vi "add channel to configuration.vi"(8 "error in":errorcluster, 10 "Modbus Module Channel.lvclass":refnum<class "Modbus Module Channel.lvclass">, 11 "Modbus Slave configuration in":refnum<class "Modbus Module configuration.lvclass">) -> (0 "error out":errorcluster, 3 "Modbus Slave configuration out":refnum<class "Modbus Module configuration.lvclass">)   [LabVIEW 2015, in "Modbus Module configuration.lvclass"]
doc: "Attempt to add Channel Input to Configuration's channel list.Channel will not be added if one with the same name already exists.\n\nPlatypus Framework 1.0.1.65\nNI Systems Engineering - National Instruments"
uses:
  Modbus Module configuration.lvclass
  module channel/Modbus Module Channel.lvclass
  <vilib>/NI/Tag Bus/tag/tag descriptor.lvclass/tag descriptor.ctl
  Modbus Module configuration.lvclass/Modbus Module configuration.ctl
  <vilib>/NI/Tag Bus/tag/tag descriptor.lvclass
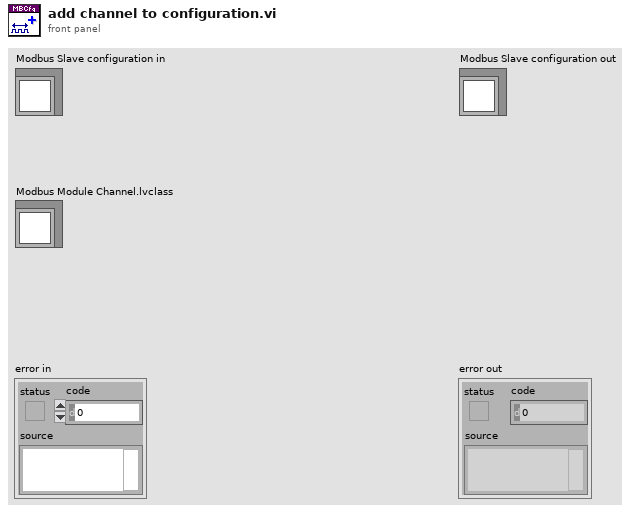
[diagram p1: front panel]
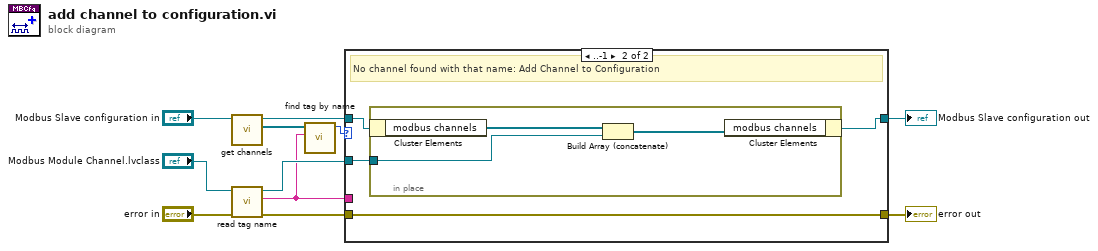
[diagram p0: block diagram]
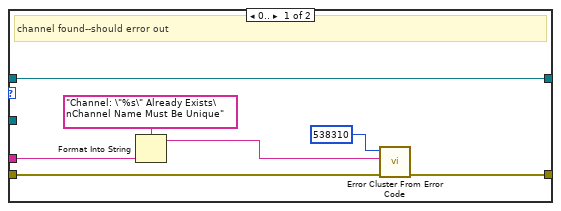
[diagram p2: hidden frame]
diagram:
  n1 = call-dynamic "get channels.vi"("Modbus Slave configuration in"="Modbus Slave configuration in") -> ("channels"=w5:refnum<class "TBM channel.lvclass">[], "Modbus Slave configuration out"=w11:refnum<class "Modbus Module configuration.lvclass">)  [unwired: 9 in]
  n2 = call <vilib>:"read tag name.vi"("error in"="error in", "system tag in"="Modbus Module Channel.lvclass") -> ("error out"=w2:errorcluster, "name"=w3:string, "system tag out"=w10:refnum<class "Modbus Module Channel.lvclass">)  [unwired: 7 in]
  n3 = call <vilib>:"find tag by name.vi"("name"=w3, "tags in"=w5) -> ("index"=w4:i32)  [unwired: 9 in]
  n4 = case shown="..-1" w4 {
    tunnel: [w18 w21] -> w8
    tunnel: w3 -> [w13 _]
    tunnel: w2 -> [w16 w21]
    tunnel: w11 -> [w15 w20]
    tunnel: w10 -> [_ w22]
    tunnel: [w15 w19] -> w7
    frame 0.. {
      # "channel found--should error out"
      n5 = Format Into String(format string="Channel: \"%s\" Already Exists\nChannel Name Must Be Unique", w13) -> (resulting string=w12:string)  [unwired: 2 in, 1 out]
      n6 = call <vilib>:"Error Cluster From Error Code.vi"("error in (no error)"=w16, "error message (\"\")"=w12, "error code (0)"=538310) -> ("error out"=w18:errorcluster)  [unwired: 6 in]
    }
    frame ..-1 {
      # "No channel found with that name: Add Channel to Configuration"
      n7 = in-place {
        in-place-border: w22 -> [w25]
        n8 = in-place-cluster #1(w20) -> ("modbus channels"=w23:refnum<class "Modbus Module Channel.lvclass">[])
        n9 = Build Array (concatenate)(w23, w25) -> (w24:refnum<class "Modbus Module Channel.lvclass">[])
        n10 = in-place-cluster #1("modbus channels"=w24) -> (w19:refnum<class "Modbus Module configuration.lvclass">)
      }
    }
  }
  "error out" <- w8
  "Modbus Slave configuration out" <- w7
